vi "RunOperation.vi"(10 "Inputs":string[](array[string]), 11 "Test in":refnum<class "Test.lvclass">) -> (1 "Output/Failure":string, 2 "CLI Process Return Code":i32, 3 "Test out":refnum<class "Test.lvclass">)   [LabVIEW 2017, in "Test.lvclass"]
uses:
  Test.lvclass
  LVUnit Test Discoverer/LVUnit Test Discoverer.lvclass
  LVUnit Test Executor/LVUnit Test Executor.lvclass
  C:/Users/pasca/Projects/Home/lvunit/Test Executor/Test Executor.lvclass
  Test.lvclass/Test.ctl
  Cobertura/Project Inspector/Project Inspector.lvclass
  C:/Users/pasca/Projects/Home/lvunit/Cobertura/Project Inspector Base/Project Inspector Base.lvclass
  Cobertura/Code Inspector/Code Inspector.lvclass
  C:/Users/pasca/Projects/Home/lvunit/Cobertura/Code Inspector Base/Code Inspector Base.lvclass
  Test Executor/Test Executor.lvclass
  Cobertura/Cobertura.lvlib
  JUnit/JUnit.lvlib
  Code Coverage/Code Coverage.lvclass
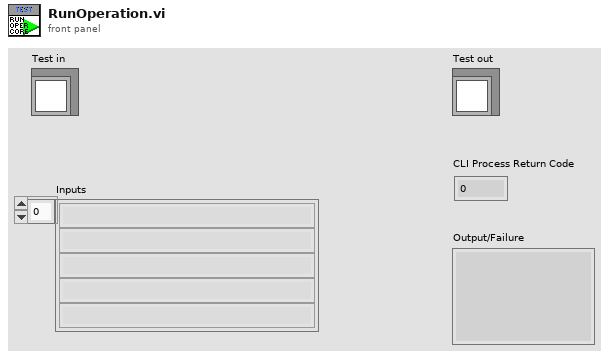
[diagram p1: front panel]
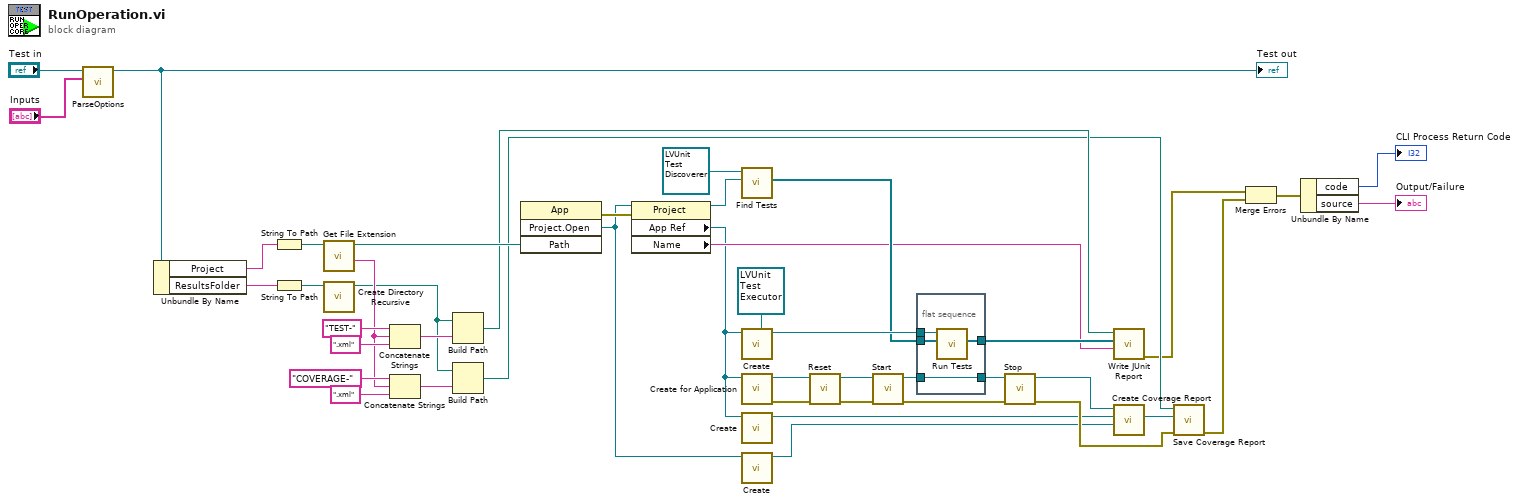
[diagram p0: block diagram]
diagram:
  n1 = call "ParseOptions.vi"("Options"="Inputs", "Test in"="Test in") -> ("Test out"=w41:refnum<class "Test.lvclass">)  [unwired: 8 in, 1 out]
  "Test out" <- w41
  n2 = Unbundle By Name(w41) -> ("Project"=w40:string, "ResultsFolder"=w38:string)
  n3 = String To Path(string=w40) -> (path=w36:path)
  n4 = String To Path(string=w38) -> (path=w37:path)
  n5 = call <vilib>:"Get File Extension.vi"("file"=w36) -> ("filename without extension"=w19:string, "dup file"=w32:path)  [unwired: 6 in, 3 out]
  n6 = call <vilib>:"Create Directory Recursive.vi"("directory"=w37) -> ("directory copy"=w17:path)  [unwired: 4 in, 2 out]
  n7 = Concatenate Strings("TEST-" ("string"), w19, ".xml" ("string")) -> (w33:string)
  n8 = Concatenate Strings("COVERAGE-" ("string"), w19, ".xml" ("string")) -> (w18:string)
  n9 = Build Path(base path=w17, name or relative path=w33) -> (appended path=w22:path)
  n10 = Build Path(base path=w17, name or relative path=w18) -> (appended path=w15:path)
  n11 = invoke class="App" method="Project.Open"("Path"=w32) -> (error out=w39:errorcluster, "Project:Open"=w2:refnum<vi>)  [unwired: 3 in, 2 out]
  n12 = property class="Project"(reference=w2, error in=w39) -> (reference out=w29:refnum<vi>, "App Ref"=w4:refnum<vi>, "Name"=w7:string)  [unwired: 1 out]
  n13 = call-dynamic "Find Tests.vi"("Project Refnum"=w29, "LVUnit Test Discoverer in"=refnum<class "LVUnit Test Discoverer.lvclass"> refnum ("LVUnit Test Discoverer")) -> ("Test Cases"=w25:refnum<class "Test Case.lvclass">[])  [unwired: 7 in, 2 out]
  n14 = call "Create.vi"("Test Executor in"=refnum<class "LVUnit Test Executor.lvclass"> refnum ("LVUnit Test Executor"), "Application"=w4) -> ("Test Executor"=w26:refnum<class "LVUnit Test Executor.lvclass">)  [unwired: 8 in, 1 out]
  n15 = call "Create for Application.vi"("Application"=w4) -> ("error out"=w8:errorcluster, "CodeCoverage out"=w27:refnum<class "Code Coverage.lvclass">)  [unwired: 9 in]
  n16 = call "Create.vi"("Application"=w4) -> ("Code Inspector"=w3:refnum<class "Code Inspector.lvclass">)  [unwired: 9 in, 1 out]
  n17 = call "Create.vi"("Project"=w2) -> ("Project Inspector"=w1:refnum<class "Project Inspector.lvclass">)  [unwired: 9 in, 1 out]
  n18 = call "Reset.vi"("error in (no error)"=w8, "CodeCoverage in"=w27) -> ("error out"=w9:errorcluster, "CodeCoverage out"=w28:refnum<class "Code Coverage.lvclass">)  [unwired: 8 in]
  n19 = call "Start.vi"("error in (no error)"=w9, "CodeCoverage in"=w28) -> ("error out"=w10:errorcluster, "CodeCoverage out"=w6:refnum<class "Code Coverage.lvclass">)  [unwired: 8 in]
  n20 = flat-sequence {
    tunnel: w26 -> [w49]
    tunnel: w25 -> [w48]
    tunnel: [w47] -> w23
    tunnel: w6 -> [w46]
    tunnel: [w46] -> w5
    frame #0 {
      n21 = call-dynamic "Run Tests.vi"("Test Cases"=w48, "LVUnit Test Executor in"=w49) -> ("Test Results"=w47:refnum<class "Test Result.lvclass">[])  [unwired: 7 in, 2 out]
    }
  }
  n22 = call "Stop.vi"("error in (no error)"=w10, "CodeCoverage in"=w5) -> ("error out"=w11:errorcluster, "CodeCoverage out"=w24:refnum<class "Code Coverage.lvclass">)  [unwired: 8 in]
  n23 = call "Write JUnit Report.vi"("Project Name"=w7, "Test Results"=w23, "File Path"=w22) -> ("error out"=w13:errorcluster)  [unwired: 8 in]
  n24 = call "Create Coverage Report.vi"("Project Inspector"=w1, "Code Inspector"=w3, "CodeCoverage in"=w24) -> ("Coverage"=w16:refnum<class "Coverage.lvclass">)  [unwired: 7 in, 1 out]
  n25 = call "Save Coverage Report.vi"("error in (no error)"=w11, "Coverage"=w16, "Path"=w15) -> ("error out"=w12:errorcluster)  [unwired: 8 in]
  n26 = Merge Errors(w13, w12) -> (w14:errorcluster)
  n27 = Unbundle By Name(w14) -> ("code"=→"CLI Process Return Code":i32, "source"=→"Output/Failure":string)
